vi "Is Feature Enabled.vi"(8 "error in":errorcluster, 11 "feature name":string) -> (0 "error out":errorcluster, 3 "feature enabled?":bool)   [LabVIEW 2019, in "grpc-lvsupport.lvlib"]
uses:
  grpc-lvsupport.lvlib
  <vilib>/Utility/error.llb/Error Cluster From Error Code.vi
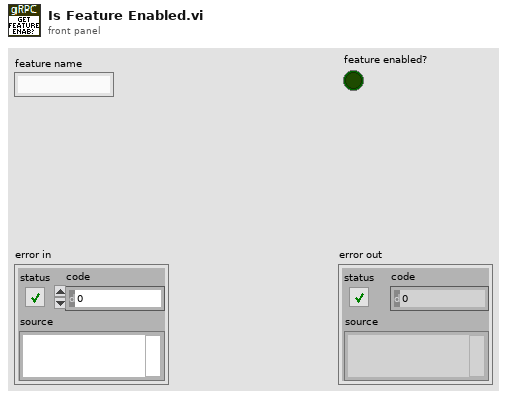
[diagram p1: front panel]
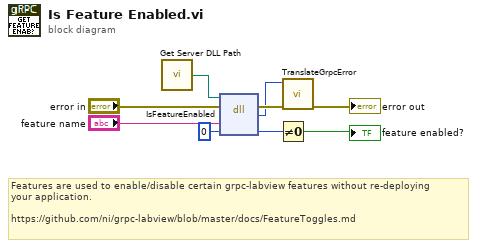
[diagram p0: block diagram]
diagram:
  # "Features are used to enable/disable certain grpc-labview features without re-deploying\nyour application.\n\nhttps://github.com/ni/grpc-labview/blob/master/docs/FeatureToggles.md"
  n1 = call "Get Server DLL Path.vi"() -> ("server dll path"=w4:path)
  n2 = dll-call lib="?" fn="IsFeatureEnabled"(path in=w4, error in="error in", "featureName"="feature name", "featureEnabled"=u8 0) -> (error out=w5:errorcluster, "return type"=w3:i32, "featureEnabled"=w1:u8)  [unwired: 2 in, 1 out]
  n3 = Not Equal To 0?(x=w1) -> (x != 0?=→"feature enabled?":bool)
  n4 = call "TranslateGrpcError.vi"("error in"=w5, "Error Code"=w3) -> ("error out"=→"error out":errorcluster)  [unwired: 9 in]
